vi "read_position_nodata__f3e8f76318.vi"(8 "error in (no error)":errorcluster, 10 "relative seconds":dbl, 11 "Refnum in":refnum<k21>) -> (0 "error out":errorcluster, 1 "String":string, 2 "data":dbl, 3 "Refnum out":refnum<k21>)   [LabVIEW 2023]
uses:
  <vilib>/DAQmx/read.llb/DAQmx Read (Analog DBL 1Chan 1Samp).vi
  <vilib>/DAQmx/miscellaneous.llb/DAQmx Fill In Error Info.vi
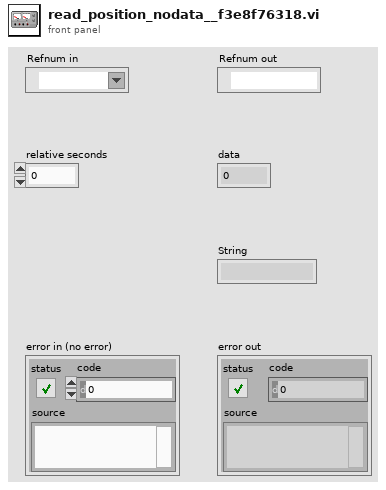
[diagram p1: front panel]
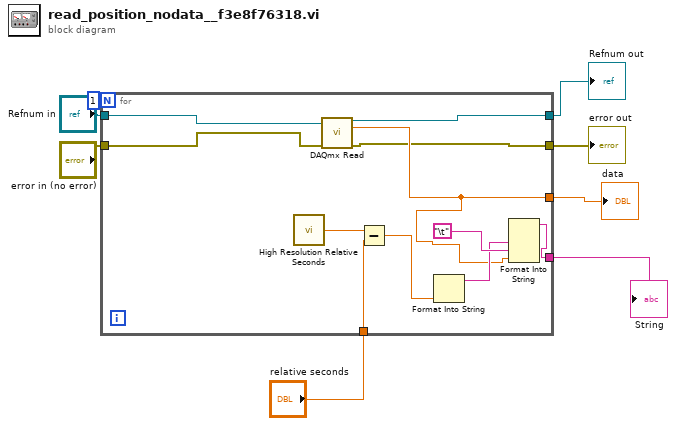
[diagram p0: block diagram]
diagram:
  n1 = for {
    N: 1 -> [_]
    tunnel: [w13] -> w7
    tunnel: [w14] -> w2
    tunnel: "relative seconds" -> [w18]
    tunnel: "Refnum in" -> [w10]
    tunnel: [w11] -> w4
    tunnel: "error in (no error)" -> [w9]
    tunnel: [w12] -> w1
    n2 = call <vilib>:"High Resolution Relative Seconds.vi"() -> ("relative seconds"=w17:dbl)
    n3 = call-poly <vilib>:"DAQmx Read.vi"("task/channels in"=w10, "error in"=w9) -> ("task out"=w11:refnum<k21>, "data"=w14:dbl, "error out"=w12:errorcluster)  [unwired: 11 in]
    n4 = Subtract(x=w17, y=w18) -> (x-y=w19:dbl)
    n5 = Format Into String(w19) -> (resulting string=w15:string)  [unwired: 3 in, 1 out]
    n6 = Format Into String(w15, "\t", w14) -> (resulting string=w13:string)  [unwired: 3 in, 1 out]
  }
  "String" <- w7
  "Refnum out" <- w4
  "data" <- w2
  "error out" <- w1
